vi "Filter Subfolders.vi"(10 "Root Path":path, 11 "Paths in":path[](array[path])) -> (3 "Paths out":path[](array[path]))   [LabVIEW 2026]
doc: "This VI removes all paths that do not reside inside the provided root path."
uses:
  <userlib>/_OpenG.lib/file/file.llb/Strip Path - Arrays__ogtk.vi
  <userlib>/_OpenG.lib/file/file.llb/openg_file.lvlib
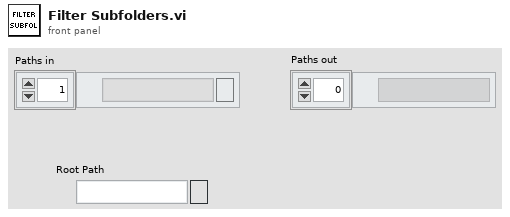
[diagram p1: front panel]
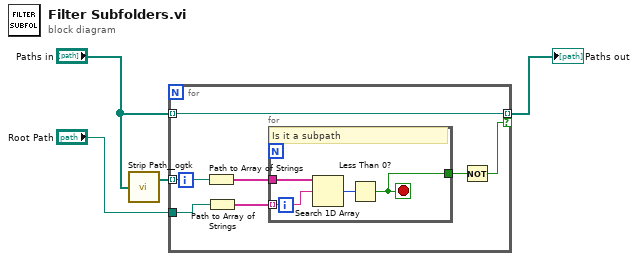
[diagram p0: block diagram]
diagram:
  n1 = call-poly <userlib>:"Strip Path__ogtk.vi"("path"="Paths in") -> ("stripped path"=w4:path[])  [unwired: 1 out]
  n2 = for {
    tunnel: w4 -> [w7] mode=indexing
    tunnel: "Root Path" -> [w11]
    tunnel: [w5] -> w1 mode=indexing if=w6
    tunnel: "Paths in" -> [w5] mode=indexing
    n3 = Path to Array of Strings(0:w7) -> (2:w10:string[])  [unwired: 1 out]
    n4 = Path to Array of Strings(0:w11) -> (2:w9:string[])  [unwired: 1 out]
    n5 = for {
      tunnel: w10 -> [w13]
      tunnel: w9 -> [w12] mode=indexing
      tunnel: [w14] -> w8
      stop <- w14 stop-if-true
      # "Is it a subpath"
      n6 = Search 1D Array(1D array=w13, element=w12) -> (index of element=w15:i32)  [unwired: 1 in]
      n7 = Less Than 0?(x=w15) -> (x < 0?=w14:bool)
    }
    n8 = Not(x=w8) -> (.not. x?=w6:bool)
  }
  "Paths out" <- w1
